vi "ZM-CP-FL-appendLine.vi"(8 "error in (no error)":errorcluster, 10 "line":string, 11 "file":path) -> (0 "error out":errorcluster)   [LabVIEW 2020, in "ZM-CP-FL-file_logger.lvlib" / "ZM-CP-FL-file_logger.lvclass"]
doc: "Appends one line plus LF to a JSON Lines file, creating the file if missing. The file is opened and closed per write, so every line is flushed."
uses:
  ZM-CP-FL-file_logger.lvclass
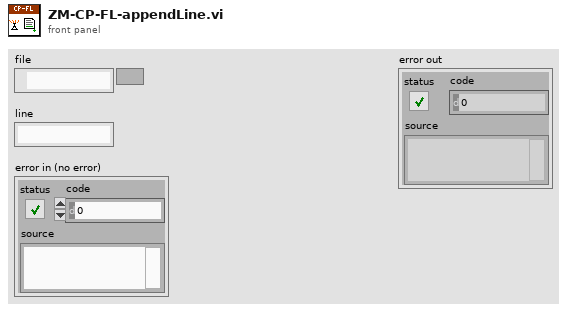
[diagram p1: front panel]
types:
  T1 = enum16{"open", "replace", "create", "open or create", "replace or create", "replace or create with confirmation"}
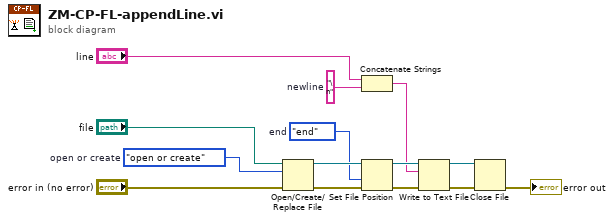
[diagram p0: block diagram]
diagram:
  w8 = enum16{"start", "end", "current"}."end"  # end
  w11 = T1."open or create"  # open or create
  w13 = "\n"  # newline
  n1 = Open/Create/Replace File(file path (use dialog)="file", error in="error in (no error)", operation (0:open)=w11) -> (refnum out=w9:refnum<file>, error out=w7:errorcluster)  [unwired: 3 in, 1 out]
  n2 = Concatenate Strings("line", w13) -> (w5:string)
  n3 = Set File Position(refnum=w9, from (0:start)=w8, error in=w7) -> (refnum out=w6:refnum<file>, error out=w4:errorcluster)  [unwired: 1 in]
  n4 = Write to Text File(file (use dialog)=w6, text=w5, error in=w4) -> (refnum out=w3:refnum<file>, error out=w2:errorcluster)  [unwired: 1 in, 1 out]
  n5 = Close File(refnum=w3, error in=w2) -> (error out=→"error out":errorcluster)  [unwired: 1 out]
